vi "func_gen_2021_ALL.vi"() -> ()   [LabVIEW 2019]
uses:
  <instrlib>/Agilent 3446X Series/Public/Data/Read (Single Point).vi
  <instrlib>/Agilent 33XXX Series/Agilent 33XXX Series.lvlib
  <instrlib>/Agilent 3446X Series/Agilent 3446X Series.lvlib
  <vilib>/Analysis/NI_AALBase.lvlib
  <instrlib>/Rohde&Schwarz RTx Oscilloscopes/Rohde&Schwarz RTx Oscilloscopes.lvlib
panel:
  out "standard deviation 2":dbl=8.042600220123908e-06 format="%0.2f"
  out "MEAN 2":i32
  out "ARRAY 2":dbl[](array[numeric])=[-0.000445167035, -0.000440579343, -0.000437663457, -0.000430911847, -0.000437185142, -0.000423927978, -0.000424408594, -0.000432868803, -0.000422637906, -0.000423852092, -0.000442083278, -0.000418949356, -0.000427140512, -0.000438994923, -0.000426889856, -0.000420278522, -0.000429614876, -0.000438923635, -0.000441154242, -0.000431873078]
  out "Waveform Graph":dbl[](graph)
  in  "Time Base Range (0.5)":dbl=0.5 caption="Time Per Record (0.5)" format="%.3e"
  in  "Channel (1) 2":i32(ring)=1 caption="Channel (1)" items=["1"=1, "2"=2, "3"=3, "4"=4, "External"=5]
  in  "Vertical Coupling (DC 1 MOhm)":i32(ring) items=["AC", "DC 50 Ohm", "DC 1 MOhm", "AC 1 MOhm", "Ground"]
  in  "Vertical Range (0.04)":dbl=0.04 format="%.3e"
  out "Measurement Result":dbl format="%^.3e"
  in  "Measurement Function (Frequency)":i32(ring)=1 items=["Frequency"=1, "Period"=2, "Peak Peak"=3, "Peak Upper"=4, "Peak Lower"=5, "Positive Pulses Count"=6, "Negative Pulses Count"=7, "Rising Edges Count"=8, "Falling Edges Count"=9, "High"=10, "Low"=11, "Amplitude"=12, "Mean Value"=13, "RMS Value"=14, "Rise Time"=15, "Falling Time"=16, "Duty Cycle Positive"=17, "Duty Cycle Negative"=18, "Pulse Width Positive"=19, "Pulse Width Negative"=20, "Cycle Mean"=21, "Cycle RMS"=22, "Standard Deviation"=23, "Delay"=26, "Phase"=27, "Burst Width"=28, "Cycle Standard Deviation"=29, "Positive Overshoot"=30, "Negative Overshoot"=31]
  out "standard deviation":dbl=8.042600220123908e-06 format="%0.2f"
  out "MEAN":i32
  out "ARRAY":dbl[](array[numeric])=[-0.000445167035, -0.000440579343, -0.000437663457, -0.000430911847, -0.000437185142, -0.000423927978, -0.000424408594, -0.000432868803, -0.000422637906, -0.000423852092, -0.000442083278, -0.000418949356, -0.000427140512, -0.000438994923, -0.000426889856, -0.000420278522, -0.000429614876, -0.000438923635, -0.000441154242, -0.000431873078]
  out "Measurement":dbl=-0.000431873078
  in  "Measurement Function (10: Voltage DC)":i32(ring)=9 items=["Continuity", "Current AC", "Current DC", "Diode", "Frequency", "Resistance 4-wire", "Period", "Resistance 2-wire", "Temperature", "Voltage AC", "Voltage DC", "Voltage DC Ratio", "Capacitance"]
  in  "Frequency (1000 Hz)":dbl=1000.0
  in  "Amplitude (1)":dbl=1.0
  in  "Waveform Function (1: Sine)":u16(ring)=1 items=["DC", "Sine", "Square", "Triangle", "Ramp", "Pulse", "Noise", "Sinc", "Negative Ramp", "Exponential Rise", "Exponential Fall", "Cardiac"]
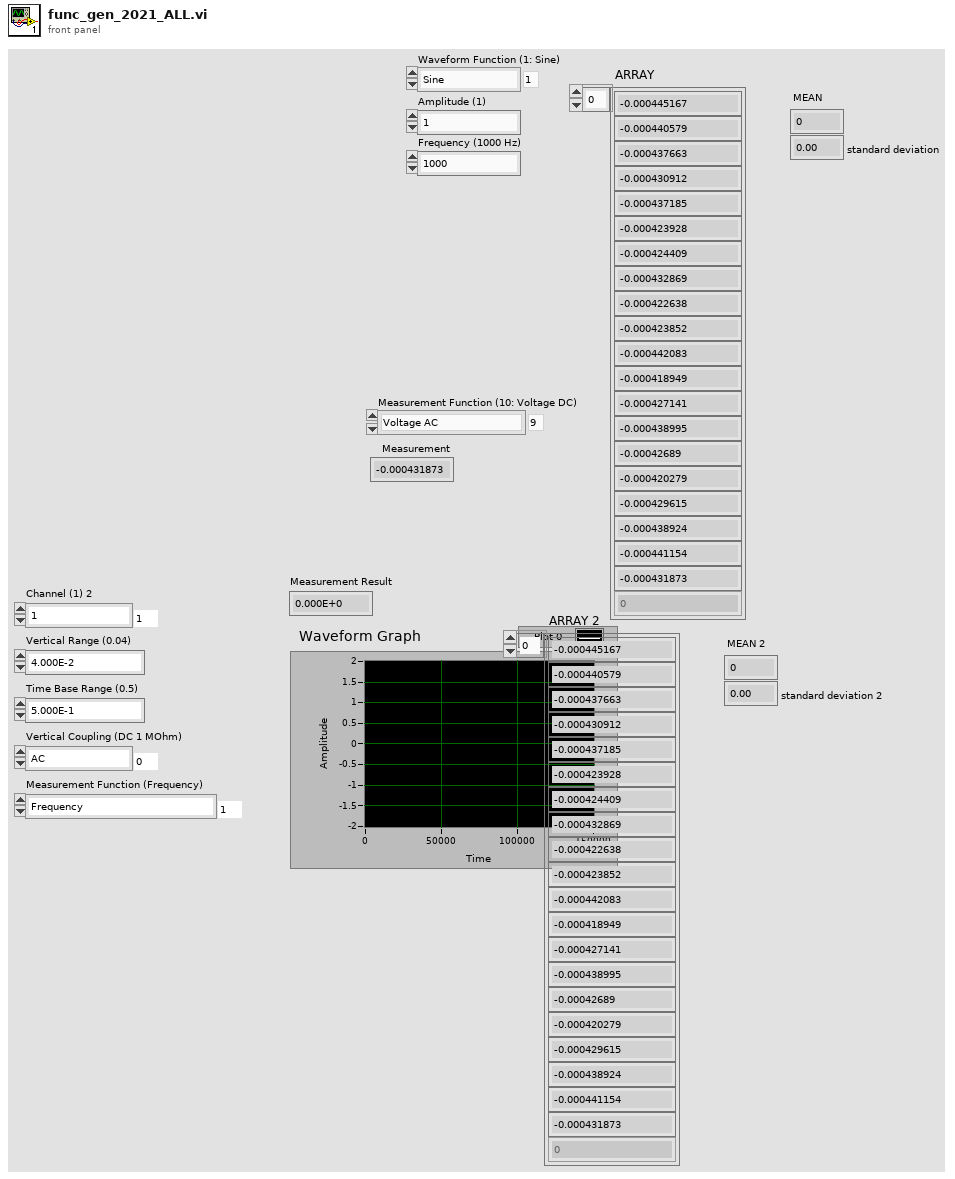
[diagram p1: front panel]
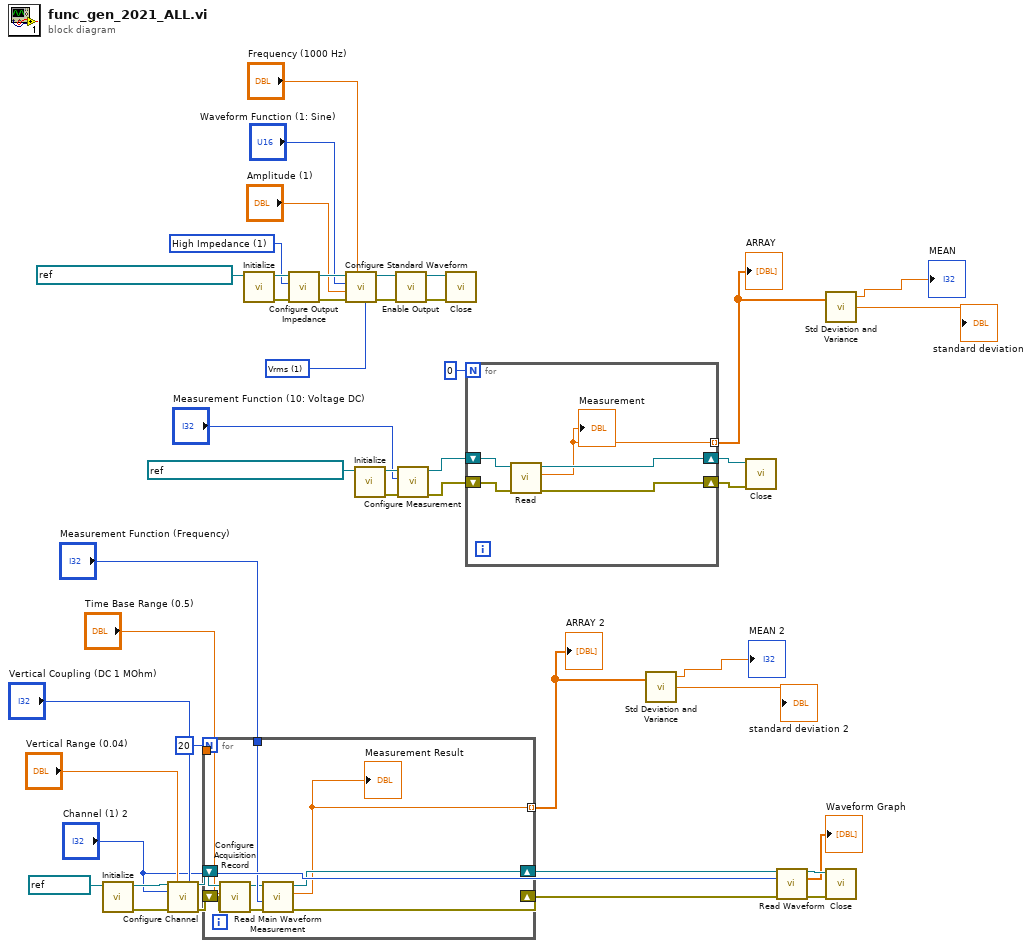
[diagram p0: block diagram]
diagram:
  w32 = u16 1 items=["Vpp", "Vrms", "dB"] ("Unit (0: Vpp)")
  w43 = u16 1 items=["50 Ohms", "High Impedance", "User Defined"] ("Impedance (0: 50 Ohms)")
  n1 = call <instrlib>:"Initialize.vi"("VISA resource name"=refnum<visa-resource-name> "Rhode") -> ("error out"=w10:errorcluster, "VISA resource name out"=w11:refnum<visa-resource-name>)  [unwired: 9 in]
  n2 = call <instrlib>:"Configure Channel.vi"("VISA resource name"=w11, "Vertical Range (0.04)"="Vertical Range (0.04)", "Vertical Coupling (DC 1 MOhm)"="Vertical Coupling (DC 1 MOhm)", "Channel (1)"="Channel (1) 2", "error in (no error)"=w10) -> ("VISA resource name out"=w9:refnum<visa-resource-name>, "error out"=w8:errorcluster)  [unwired: 9 in]
  n3 = for {
    N: 20 -> [_]
    tunnel: "Measurement Function (Frequency)" -> [w52]
    tunnel: "Time Base Range (0.5)" -> [w47]
    shift-right: [w54] -> w18
    shift-left: w9 -> [w51]
    shift-right: [w53] -> w17
    shift-left: w8 -> [w50]
    tunnel: [w46] -> w1 mode=indexing
    n4 = call <instrlib>:"Configure Acquisition Record.vi"("error in (no error)"=w50, "Time Per Record (0.5)"=w47, "VISA resource name"=w51) -> ("error out"=w49:errorcluster, "VISA resource name out"=w48:refnum<visa-resource-name>)  [unwired: 7 in]
    n5 = call <instrlib>:"Read Main Waveform Measurement.vi"("error in (no error)"=w49, "Measurement Function (Frequency)"=w52, "VISA resource name"=w48) -> ("error out"=w53:errorcluster, "Measurement Result"=w46:dbl, "VISA resource name out"=w54:refnum<visa-resource-name>)  [unwired: 6 in]
    "Measurement Result" <- w46
  }
  "ARRAY 2" <- w1
  n6 = call <instrlib>:"Initialize.vi"("VISA resource name"=refnum<visa-resource-name> "TCPIP0::192.168.2.3::inst0::INSTR") -> ("error out"=w44:errorcluster, "VISA resource name out"=w45:refnum<visa-resource-name>)  [unwired: 9 in]
  n7 = call <instrlib>:"Configure Output Impedance.vi"("error in (no error)"=w44, "Impedance (0: 50 Ohms)"=w43, "VISA resource name"=w45) -> ("error out"=w41:errorcluster, "VISA resource name out"=w42:refnum<visa-resource-name>)  [unwired: 7 in]
  n8 = call <instrlib>:"Configure Standard Waveform.vi"("Unit (0: Vpp)"=w32, "Frequency (1000 Hz)"="Frequency (1000 Hz)", "error in (no error)"=w41, "Amplitude (1)"="Amplitude (1)", "Waveform Function (1: Sine)"="Waveform Function (1: Sine)", "VISA resource name"=w42) -> ("error out"=w36:errorcluster, "VISA resource name out"=w35:refnum<visa-resource-name>)  [unwired: 4 in]
  n9 = call <instrlib>:"Initialize.vi"("VISA resource name"=refnum<visa-resource-name> "TCPIP0::192.168.2.4::inst0::INSTR") -> ("error out"=w31:errorcluster, "VISA resource name out"=w28:refnum<visa-resource-name>)  [unwired: 9 in]
  n10 = call <instrlib>:"Enable Output.vi"("error in (no error)"=w36, "VISA resource name"=w35) -> ("error out"=w33:errorcluster, "VISA resource name out"=w34:refnum<visa-resource-name>)  [unwired: 8 in]
  n11 = call <instrlib>:"Configure Measurement.vi"("error in (no error)"=w31, "Measurement Function (10: Voltage DC)"="Measurement Function (10: Voltage DC)", "VISA resource name"=w28) -> ("error out"=w25:errorcluster, "VISA resource name out"=w26:refnum<visa-resource-name>)  [unwired: 7 in]
  n12 = call <instrlib>:"Close.vi"("error in (no error)"=w33, "VISA resource name"=w34) -> ()  [unwired: 9 in, 1 out]
  n13 = for {
    N: 0 -> [_]
    shift-right: [w58] -> w29
    shift-left: w26 -> [w57]
    shift-right: [w59] -> w30
    shift-left: w25 -> [w56]
    tunnel: [w55] -> w23 mode=indexing
    n14 = call-poly <instrlib>:"Read.vi"("error in (no error)"=w56, "VISA resource name"=w57) -> ("error out"=w59:errorcluster, "Measurement"=w55:dbl, "VISA resource name out"=w58:refnum<visa-resource-name>)  [unwired: 7 in]
    "Measurement" <- w55
  }
  "ARRAY" <- w23
  n15 = call <vilib>:"Std Deviation and Variance.vi"("X"=w1) -> ("mean"=→"MEAN 2":dbl, "standard deviation"=→"standard deviation 2":dbl)  [unwired: 1 in, 1 out]
  n16 = call <instrlib>:"Close.vi"("error in (no error)"=w30, "VISA resource name"=w29) -> ()  [unwired: 9 in, 1 out]
  n17 = call <instrlib>:"Read Waveform.vi"("VISA resource name"=w18, "Channel (1)"="Channel (1) 2", "error in (no error)"=w17) -> ("VISA resource name out"=w15:refnum<visa-resource-name>, "Waveform Array"=→"Waveform Graph":dbl[], "error out"=w14:errorcluster)  [unwired: 7 in, 3 out]
  n18 = call <vilib>:"Std Deviation and Variance.vi"("X"=w23) -> ("mean"=→"MEAN":dbl, "standard deviation"=→"standard deviation":dbl)  [unwired: 1 in, 1 out]
  n19 = call <instrlib>:"Close.vi"("error in (no error)"=w14, "VISA resource name"=w15) -> ()  [unwired: 9 in, 1 out]
